vi "Function Name String Constant Label--constant.vi"() -> (3 "Function Name String Constant Label":string)   [LabVIEW 2026]
doc: "This constant defines the label of the string constant that defines the function name in the template VI."
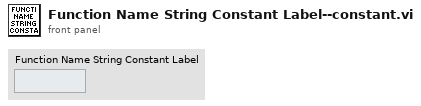
[diagram p1: front panel]
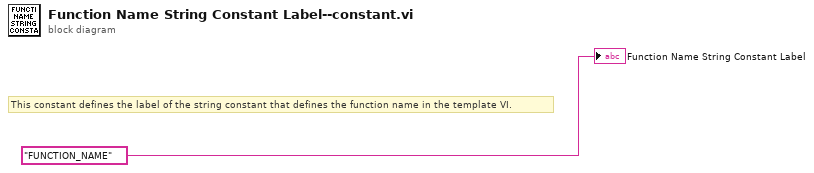
[diagram p0: block diagram]
diagram:
  # "This constant defines the label of the string constant that defines the function name in the template VI."
  "Function Name String Constant Label" <- "FUNCTION_NAME" ("Function Name String Constant Label")
